vi "RemoteVI Target Geometry.vi"(0 "VI":refnum<vi>, 5 "window":u64, 11 "error in":errorcluster) -> (4 "geo":T1, 6 "hWnd":u64, 8 "origin":cluster{"x":i32, "y":i32}, 15 "error out":errorcluster)   [LabVIEW 2020, in "RemoteVI.lvlib"]
doc: "Where the shared window is on screen, for VI or for a window of any process. window 0: the front panel window of VI (RemoteVI Get Panel Geometry.vi, VI Server). Otherwise window is the shared window itself (a window target, e.g. a panel of another LabVIEW process or another program): the frame is its client area, so geo.panelX/panelY and clientX/clientY are both the client-area origin on screen (-ScreenToClient(0,0)) and the panel starts at the frame's origin (origin 0,0); no VI Server call."
uses:
  RemoteVI.lvlib
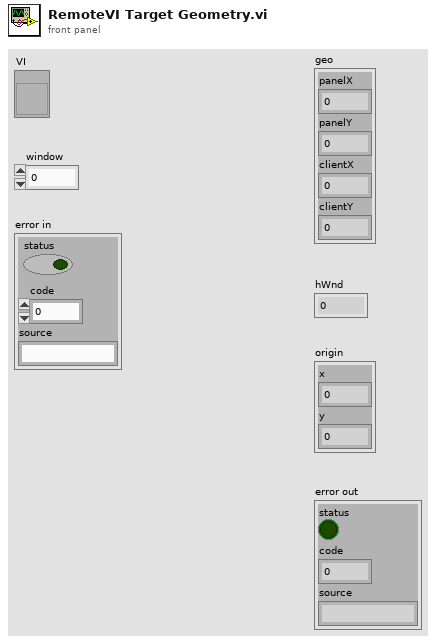
[diagram p1: front panel]
types:
  T1 = cluster{"panelX":i32, "panelY":i32, "clientX":i32, "clientY":i32}
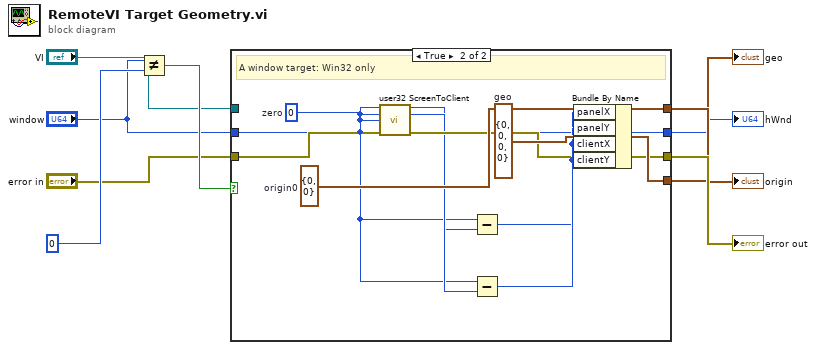
[diagram p0: block diagram]
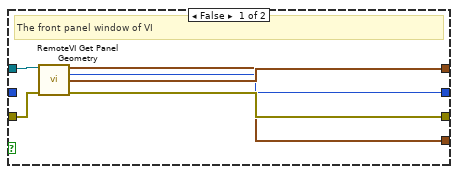
[diagram p2: hidden frame]
diagram:
  n1 = Not Equal?(x="window", y=u64 0) -> (x != y?=w5:bool)
  n2 = case shown="True" w5 {
    tunnel: "VI" -> [w10 _]
    tunnel: "window" -> [_ w16]
    tunnel: "error in" -> [w11 w17]
    tunnel: [w14 w26] -> w8
    tunnel: [w13 w16] -> w7
    tunnel: [w15 w21] -> w9
    tunnel: [w12 w25] -> w6
    frame False {
      # "The front panel window of VI"
      n3 = call "RemoteVI Get Panel Geometry.vi"("VI"=w10, "error in"=w11) -> ("geo"=w12:T1, "hWnd"=w13:u64, "origin"=w14:cluster{"x":i32, "y":i32}, "error out"=w15:errorcluster)  [unwired: 10 in]
    }
    frame True {
      w26 = cluster{"x":i32, "y":i32} {"x"=0, "y"=0}  # origin0
      w24 = T1 {"panelX"=0, "panelY"=0, "clientX"=0, "clientY"=0}  # geo
      w18 = 0  # zero
      # "A window target: Win32 only"
      n4 = call "user32 ScreenToClient.vi"("hWnd"=w16, "Screen X"=w18, "Screen Y"=w18, "error in (no error)"=w17) -> ("Client X"=w19:i32, "Client Y"=w20:i32, "error out"=w21:errorcluster)  [unwired: 8 in, 1 out]
      n5 = Subtract(x=w18, y=w19) -> (x-y=w22:i32)
      n6 = Subtract(x=w18, y=w20) -> (x-y=w23:i32)
      n7 = Bundle By Name(cluster=w24, "panelX"=w22, "panelY"=w23, "clientX"=w22, "clientY"=w23) -> (w25:T1)
    }
  }
  "geo" <- w6
  "hWnd" <- w7
  "origin" <- w8
  "error out" <- w9
